vi "05c-multifunc_external-server.vi"() -> ()   [LabVIEW 2018, in "LV2Julia_examples.lvlib"]
uses:
  LV2Julia_examples.lvlib
  LV2Julia_core/VIs/Server or client state.ctl
  LV2Julia_core/VIs/detailed error info.ctl
  LV2Julia_core/VIs/StackFrame.ctl
  LV2Julia_core/VIs/Commands.ctl
  88ada97c-421d-418d-a763-307c6da0fd18.vi
  1e32e5d8-80f1-4661-9552-ce4369739336.vi
  f9c51bc2-fc6e-407e-bb72-37bc6f45ead0.vi
  <vilib>/Utility/High Resolution Relative Seconds.vi
  1e32e5d8-80f1-4661-9552-ce4369739336.vi/181debbd-4e55-4beb-9bb4-56b9b9eb0aec.vi
  1e32e5d8-80f1-4661-9552-ce4369739336.vi/181debbd-4e55-4beb-9bb4-56b9b9eb0aec.vi/2e64d928-ac4b-415e-9a94-a528e175af31.vi
  1e32e5d8-80f1-4661-9552-ce4369739336.vi/181debbd-4e55-4beb-9bb4-56b9b9eb0aec.vi/b7533af2-aee6-49d9-9c84-16d86a9323b8.vi
  1e32e5d8-80f1-4661-9552-ce4369739336.vi/181debbd-4e55-4beb-9bb4-56b9b9eb0aec.vi/b8f26e5b-04e5-4f84-be41-7f53a8d6f60b.vi
  LV2Julia_core/VIs/jl-scripts path.vi
  LV2Julia_core/VIs/check ID validity.vi
  LV2Julia_core/VIs/bindata_descr to JSON.vi
  LV2Julia_core/VIs/check cluster field names.vi
  LV2Julia_core/VIs/concat JSON.vi
  LV2Julia_core/VIs/build request.vi
  LV2Julia_core/VIs/Parse server response.vi
  LV2Julia_core/VIs/log jl exceptions.vi
  LV2Julia_core/LV2Julia_core.lvlib
panel:
  in  "execution control pages":enum32{"Start", "go - test"}(tab)
  in  "go":bool caption="go (Julia Server started externally)"
  in  "Start with Julia":bool caption="Start Julia Server and go"
  in  "ZMQ endpoint":string="tcp://127.0.0.1:5555"
  in  "stop this VI only":bool
  in  "stop both this VI and Julia Server":bool
  in  "operation":T1(radio)
  in  "operands":cluster{"x":dbl, "y":dbl}={"x"=2.0, "y"=2.0}
  in  "next":bool
  out "result":dbl=nan
  out "detailed error info":T2
  out "current error":errorcluster
  out "final error":errorcluster
  out "short err code":u8
  out "call duration (ms)":dbl format="%#.2f"
  out "ZMQ timeout":bool
  out "Julia script file path":path
  out "temporary script path":path
  out "Jl Server state":T4
  # "tcp://127.0.0.1:5555 \nfor local Julia Server\n\nFor a Julia Server running on a separate computer,  you probably must use an IPv4 address in numeric form (not a DNS name) - see https://stackoverflow.com/questions/6024003/why-doesnt-zeromq-work-on-localhost.\n\nFor instructions how to properly start the corresponding Julia script, see \n05-on_external_server.jl file in the jl-scripts folder.\n\nThe ZMQ endpoint control only used if Julia Server is not being started by this VI."
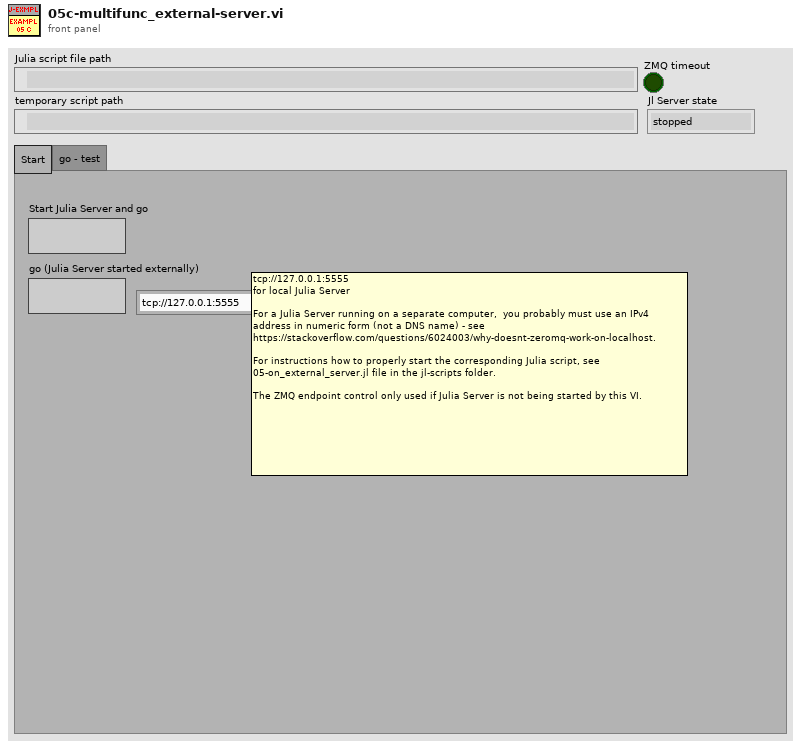
[diagram p1: front panel]
types:
  T1 = enum32{"add", "subtract", "multiply", "divide", "conquer"}
  T2 = typedef "LV2Julia_core.lvlib/detailed error info.ctl" = cluster{"exception_or_info":string, "trace":T3[]}
  T3 = typedef "LV2Julia_core.lvlib/StackFrame.ctl" = cluster{"frame_summary":string, "func":string, "linfo":string, "file":string, "line":i32, "pointer":u64, "from_c":bool, "inlined":bool}
  T4 = typedef "LV2Julia_core.lvlib/Server or client state.ctl" = enum16{"stopped", "running", "unknown"}
  T5 = typedef "LV2Julia_core.lvlib/Commands.ctl" = enum16{"Start Jl-server & Init LV-client", "Send request & Get response ", "Stop Jl-server & Cleanup LV-client", "Cleanup LV-client", "Start Jl-server", "Stop Jl-server", "Init LV-Client", "Cleanup LV-Client", "(not allowed)", "Set LV Client state", "Set Jl Server state", "set ZMQ timeout", "read ZMQ timeout", "read-out state"}
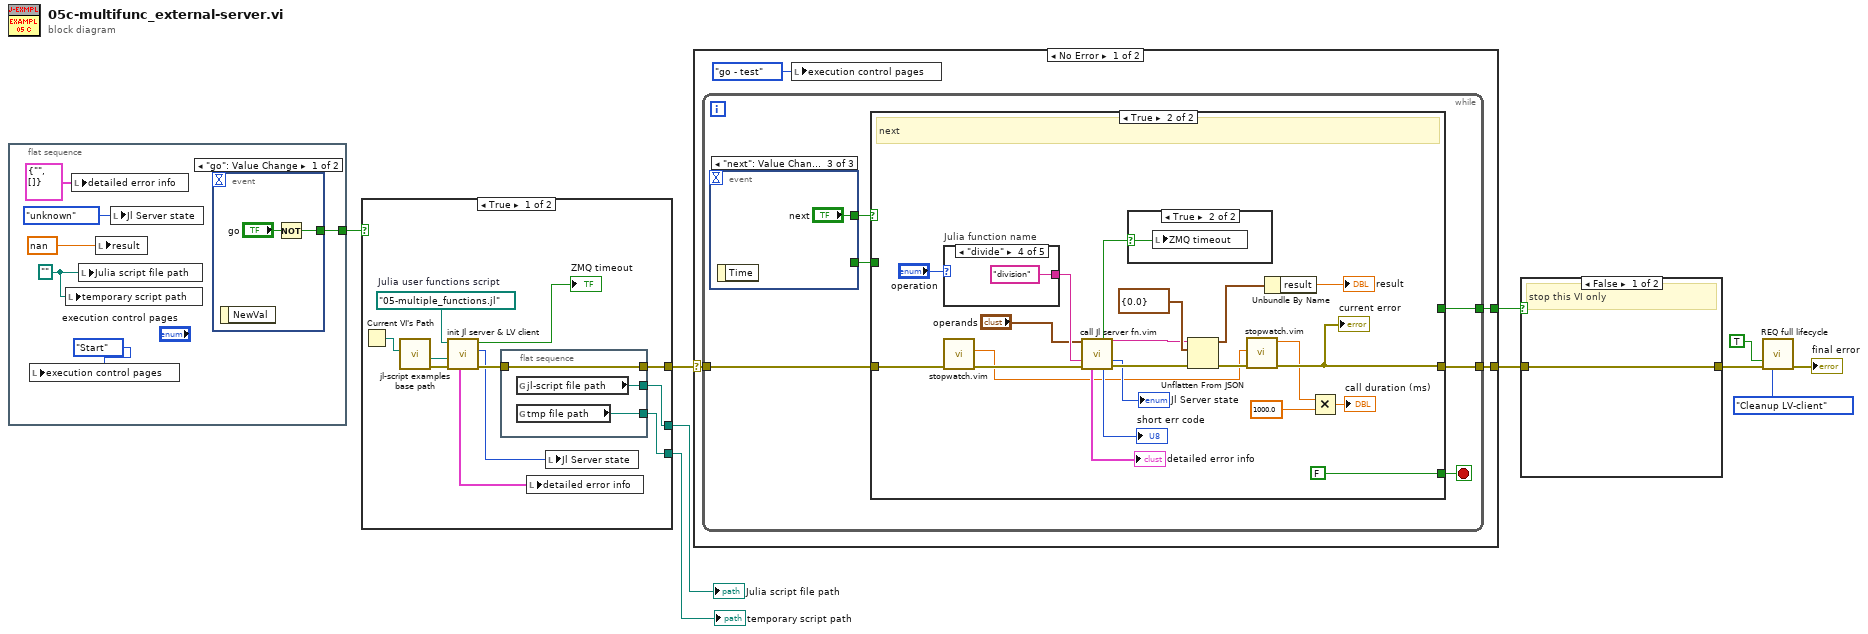
[diagram p0: block diagram]
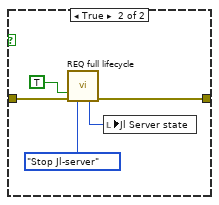
[diagram p2: hidden frame]
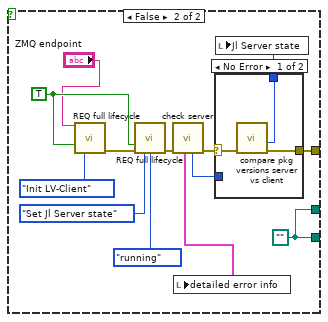
[diagram p3: hidden frame]
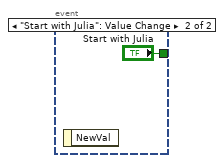
[diagram p5: hidden frame]
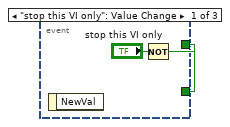
[diagram p6: hidden frame]
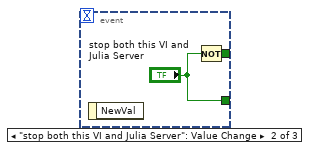
[diagram p7: hidden frame]
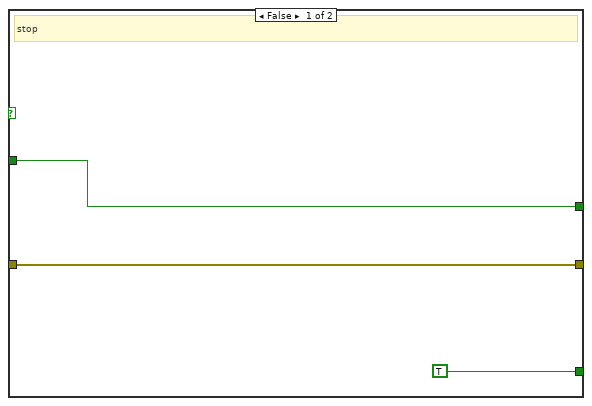
[diagram p8: hidden frame]
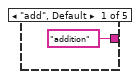
[diagram p9: hidden frame]
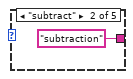
[diagram p10: hidden frame]
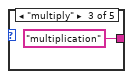
[diagram p11: hidden frame]
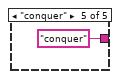
[diagram p12: hidden frame]
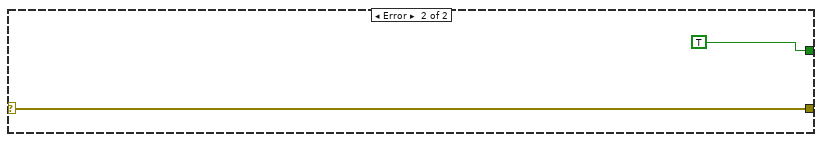
[diagram p14: hidden frame]
diagram:
  n1 = flat-sequence {
    tunnel: [w11] -> w3
    frame #0 {
      w13 = path ""
      n2 = local write "execution control pages"(enum32{"Start", "go - test"}."Start" ("execution control pages")) -> ()
      n3 = local write "temporary script path"(w13) -> ()
      n4 = local write "detailed error info"(T2 {"exception_or_info"="", "trace"=[]} ("detailed error info")) -> ()
      n5 = local write "Julia script file path"(w13) -> ()
      n6 = local write "result"(nan ("Server response")) -> ()
      n7 = local write "Jl Server state"(Server_or_client_state."unknown" ("Jl Server state out")) -> ()
      n8 = event shown="[0] \"go\": Value Change" {
        selector: _ -> [_ _]
        dyn-events: _ -> [_ _]
        timeout: _ -> [_ _]
        tunnel: [w17 "Start with Julia"] -> w11
        event "go": Value Change {
          n9 = event-data() -> ()  [unwired: 1 in, 1 out]
          n10 = Not(x="go") -> (.not. x?=w17:bool)
        }
        event "Start with Julia": Value Change {
          n11 = event-data() -> ()  [unwired: 1 in, 1 out]
        }
      }
    }
  }
  n12 = case shown="True" w3 {
    tunnel: [w30 w38] -> w6
    tunnel: [w29 w40] -> w4
    tunnel: [w28 w40] -> w5
    frame True {
      w22 = path "05-multiple_functions.jl"  # Julia user functions script
      n13 = Current VI's Path() -> (path=w26:path)
      n14 = call "jl-script examples base path.vi"("calling example VI path"=w26) -> ("error out"=w25:errorcluster, "jl-script-examples base path"=w24:path)  [unwired: 9 in]
      n15 = call "init Jl server & LV client.vi"("error in (no error)"=w25, "Base path (not a path)"=w24, "Julia user functions script"=w22) -> ("error out"=w27:errorcluster, "Jl Server state out"=w23:T4, "timeout?"=→"ZMQ timeout":bool, "detailed error info"=w20:T2)  [unwired: 3 in, 2 out]
      n16 = flat-sequence {
        tunnel: [w33] -> w30
        tunnel: w27 -> [w33]
        tunnel: [w32] -> w29
        tunnel: [w31] -> w28
        frame #0 {
          n17 = global read "jl-scripts path.vi" "jl-script file path"() -> (w32:path)
          n18 = global read "jl-scripts path.vi" "tmp file path"() -> (w31:path)
        }
      }
      n19 = local write "detailed error info"(w20) -> ()
      n20 = local write "Jl Server state"(w23) -> ()
    }
    frame False {
      w40 = path ""
      w44 = TRUE ("Force command")
      n21 = call "REQ full lifecycle.vi"("ZMQ endpoint"="ZMQ endpoint", "Force command"=w44, "command"=Commands."Init LV-Client") -> ("error out"=w42:errorcluster)  [unwired: 6 in, 6 out]
      n22 = call "REQ full lifecycle.vi"("Force command"=w44, "error in"=w42, "command"=Commands."Set Jl Server state", "Jl Server state in"=Server_or_client_state."running") -> ("error out"=w41:errorcluster)  [unwired: 5 in, 6 out]
      n23 = call "check server.vi"("error in"=w41) -> ("error out"=w39:errorcluster, "Jl Server state out"=w37:T4, "detailed error info"=w34:T2)  [unwired: 6 in, 2 out]
      n24 = local write "detailed error info"(w34) -> ()
      n25 = case shown="No Error" w39 {
        selector: w39 -> [w49 w51]
        tunnel: [w48 w51] -> w38
        tunnel: [w47 w50] -> w35
        tunnel: w37 -> [_ w50]
        frame No Error {
          n26 = call "compare pkg versions server vs client.vi"("error in (no error)"=w49) -> ("error out"=w48:errorcluster, "Jl Server state out"=w47:T4)  [unwired: 5 in, 4 out]
        }
        frame Error {
        }
      }
      n27 = local write "Jl Server state"(w35) -> ()
    }
  }
  "temporary script path" <- w5
  "Julia script file path" <- w4
  n28 = case shown="No Error" w6 {
    selector: w6 -> [w54 w98]
    tunnel: [w55 w98] -> w10
    tunnel: [w52 TRUE ("stop both this VI and Julia Server")] -> w1
    frame No Error {
      n29 = while {
        tunnel: w54 -> [w60]
        tunnel: [w61] -> w55
        tunnel: [w56] -> w52
        stop <- w58 stop-if-true
        n30 = event shown="[2] \"next\": Value Change" {
          selector: _ -> [_ _ _]
          dyn-events: _ -> [_ _ _]
          timeout: _ -> [_ _ _]
          tunnel: [w62 w65 "next"] -> w59
          tunnel: [w62 "stop both this VI and Julia Server" _] -> w57
          event "stop this VI only": Value Change {
            n31 = event-data() -> ()  [unwired: 1 in, 1 out]
            n32 = Not(x="stop this VI only") -> (.not. x?=w62:bool)
          }
          event "stop both this VI and Julia Server": Value Change {
            n33 = event-data() -> ()  [unwired: 1 in, 1 out]
            n34 = Not(x="stop both this VI and Julia Server") -> (.not. x?=w65:bool)
          }
          event "next": Value Change {
            n35 = event-data() -> ()  [unwired: 1 in, 1 out]
          }
        }
        n36 = case shown="True" w59 {
          tunnel: [w69 w72] -> w61
          tunnel: w60 -> [w69 w75]
          tunnel: [TRUE ("stop this VI only") FALSE ("stop this VI only")] -> w58
          tunnel: w57 -> [w67 _]
          tunnel: [w67 _] -> w56
          frame False {
            # "stop"
          }
          frame True {
            # "next"
            n37 = case "Julia function name" shown="\"divide\"" "operation" {
              tunnel: ["addition" "subtraction" "multiplication" "division" "conquer"] -> w84
              frame "add", Default {
              }
              frame "subtract" {
              }
              frame "multiply" {
              }
              frame "divide" {
              }
              frame "conquer" {
              }
            }
            n38 = call "stopwatch.vim"("anything in"=w75) -> ("copy of anything out"=w74:errorcluster, "current timepoint"=w71:dbl)  [unwired: 8 in, 1 out]
            n39 = call "call Jl server fn.vim"("Arguments 1"="operands", "fun2call"=w84, "error in (no error)"=w74) -> ("timeout?"=w81:bool, "JSON received"=w80:string, "Jl Server state out"=→"Jl Server state":T4, "detailed error info"=→"detailed error info":T2, "return code"=→"short err code":u8, "error out"=w85:errorcluster)  [unwired: 6 in, 1 out]
            n40 = case shown="True" w81 {
              selector: w81 -> [_ w96]
              frame False {
              }
              frame True {
                n41 = local write "ZMQ timeout"(w96) -> ()
              }
            }
            n42 = Unflatten From JSON(JSON string=w80, type and defaults=cluster{"result":dbl} {"result"=0.0} ("parsed response"), error in (no error)=w85) -> (value=w89:cluster{"result":dbl}, error out=w73:errorcluster)  [unwired: 4 in]
            n43 = call "stopwatch.vim"("anything in"=w73, "prev timepoint (0)"=w71) -> ("copy of anything out"=w72:errorcluster, "delta t (s)"=w70:dbl)  [unwired: 7 in, 1 out]
            "current error" <- w72
            n44 = Unbundle By Name(w89) -> ("result"=→"result":dbl)
            n45 = Multiply(x=w70, y=1000.0) -> (x*y=→"call duration (ms)":dbl)
          }
        }
      }
      n46 = local write "execution control pages"(enum32{"Start", "go - test"}."go - test" ("execution control pages")) -> ()
    }
    frame Error {
    }
  }
  n47 = case shown="False" w1 {
    tunnel: w10 -> [w99 w104]
    tunnel: [w99 w102] -> w9
    frame False {
      # "stop this VI only"
    }
    frame True {
      n48 = call "REQ full lifecycle.vi"("Force command"=TRUE, "error in"=w104, "command"=Commands."Stop Jl-server") -> ("Jl Server state out"=w101:T4, "error out"=w102:errorcluster)  [unwired: 6 in, 5 out]
      n49 = local write "Jl Server state"(w101) -> ()
    }
  }
  n50 = call "REQ full lifecycle.vi"("Force command"=TRUE, "error in"=w9, "command"=Commands."Cleanup LV-client") -> ("error out"=→"final error":errorcluster)  [unwired: 6 in, 6 out]
